vi "Bridge_Read_Status.vi"(8 "error in (no error)":errorcluster={"status"=FALSE, "code"=0, "source"="\"\""}, 10 "hardware status":string, 11 "Lease table":string) -> (0 "error out":errorcluster={"status"=FALSE, "code"=0, "source"="\"\""}, 2 "status ok":bool, 3 "ResourceStatus snapshot":string)   [LabVIEW 2026]
doc: "INTENT: Report resource ownership and health. LOGIC: Provide supervisor/Host view of owner, commanded mode, last ACK and fault block."
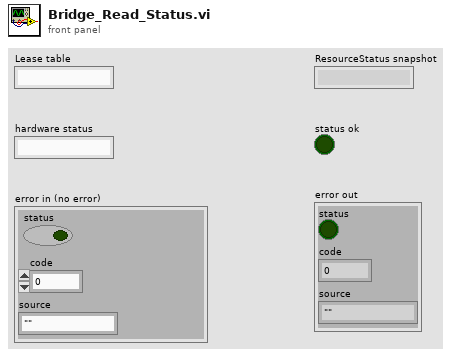
[diagram p1: front panel]
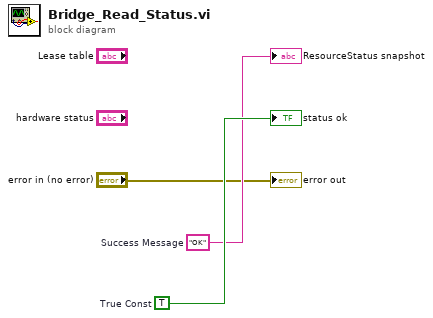
[diagram p0: block diagram]
diagram:
  w3 = TRUE  # True Const
  w2 = "OK"  # Success Message
  "ResourceStatus snapshot" <- w2
  "status ok" <- w3
  "error out" <- "error in (no error)"
